vi "ConvertDefinitionToRing.vi"() -> ()   [LabVIEW 2020, in "CTI-Tools.lvlib"]
uses:
  CTI-Tools.lvlib
  <vilib>/Utility/error.llb/Trim Whitespace One-Sided.vi
panel:
  out "error out":errorcluster
  in  "Registers":u16(ring) items=["M5_8SERVOS2_MODE_INPUT  ", "M5_8SERVOS2_MODE_OUTPUT ", "M5_8SERVOS2_MODE_ADC    ", "M5_8SERVOS2_MODE_SERVO  ", "M5_8SERVOS2_MODE_RGB    ", "M5_8SERVOS2_MODE_PWM    "]
  in  "String":string
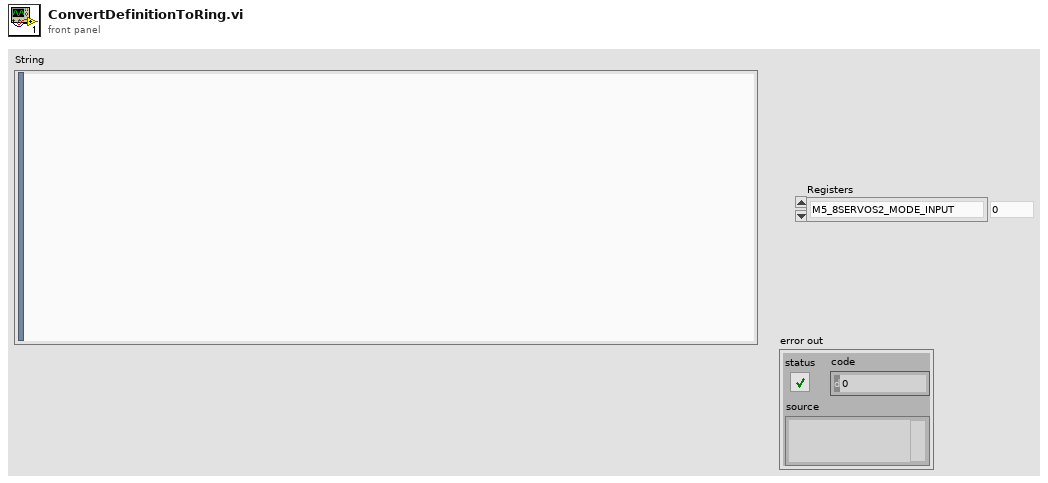
[diagram p1: front panel]
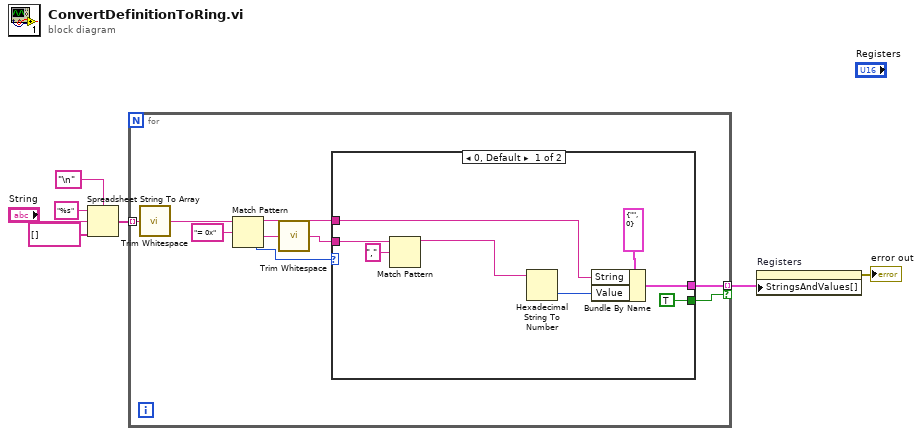
[diagram p0: block diagram]
diagram:
  n1 = Spreadsheet String To Array(delimiter (Tab)="\n", format string="%s", spreadsheet string="String", array type (2D Dbl)=string[] []) -> (array=w3:string[])
  n2 = for {
    tunnel: w3 -> [w16] mode=indexing
    tunnel: [w13] -> w2 mode=indexing if=w11
    n3 = call <vilib>:"Trim Whitespace.vi"("string"=w16) -> ("trimmed string"=w10:string)  [unwired: 1 in]
    n4 = Match Pattern(string=w10, regular expression="= 0x") -> (before substring=w8:string, after substring=w14:string, offset past match=w12:i32)  [unwired: 1 in, 1 out]
    n5 = call <vilib>:"Trim Whitespace.vi"("string"=w14) -> ("trimmed string"=w9:string)  [unwired: 1 in]
    n6 = case shown="0, Default" w12 {
      tunnel: w9 -> [w24 _]
      tunnel: [w20 _] -> w13
      tunnel: [TRUE _] -> w11
      tunnel: w8 -> [w18 _]
      frame 0, Default {
        n7 = Match Pattern(string=w24, regular expression=",") -> (before substring=w17:string)  [unwired: 1 in, 3 out]
        n8 = Hexadecimal String To Number(string=w17) -> (number=w21:u32)  [unwired: 2 in, 1 out]
        n9 = Bundle By Name(cluster=cluster{"String":string, "Value":u16} {"String"="", "Value"=0}, "String"=w18, "Value"=w21) -> (w20:cluster{"String":string, "Value":u16})
      }
      frame -1 {
      }
    }
  }
  n10 = property on="Registers" class="Ring (strict)"("StringsAndValues[]"=w2) -> (error out=→"error out":errorcluster)  [unwired: 2 in, 1 out]
